vi "module information (FPGA interface).vi"(8 "error in":errorcluster, 10 "Module":u16, 11 "Refnum in":refnum<k20>) -> (0 "error out":errorcluster, 2 "Module Information":T1 {"product ID" format="%.0x"}, 3 "Refnum out":refnum<k20>)   [LabVIEW 2014, in "SMI.lvlib" / "C Series Module.lvclass"]
uses:
  C Series Module.lvclass
  Module/module information.ctl
  <vilib>/Utility/error.llb/Error Cluster From Error Code.vi
  <vilib>/rvi/errors/niLvFpgaAdjustHostInterfaceError.vi
  <vilib>/rvi/interface/nirviReadWriteControl/nirviReadWriteControl.xnode
  <vilib>/ErrorRing/Error Ring.xnode
  Module/Module.lvclass
  NiFpgaLv.dll
  <vilib>/rvi/interface/Simulation/niFpgaSimulationCallBeginRW.vi
  SMI.lvlib
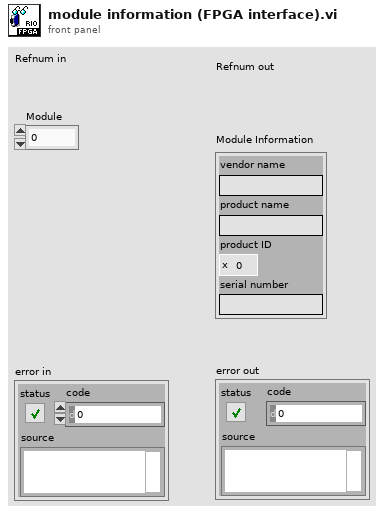
[diagram p1: front panel]
types:
  T1 = typedef "SMI.lvlib/Module.lvclass/module information.ctl" = cluster{"vendor name":string, "product name":string, "product ID":u16, "serial number":string}
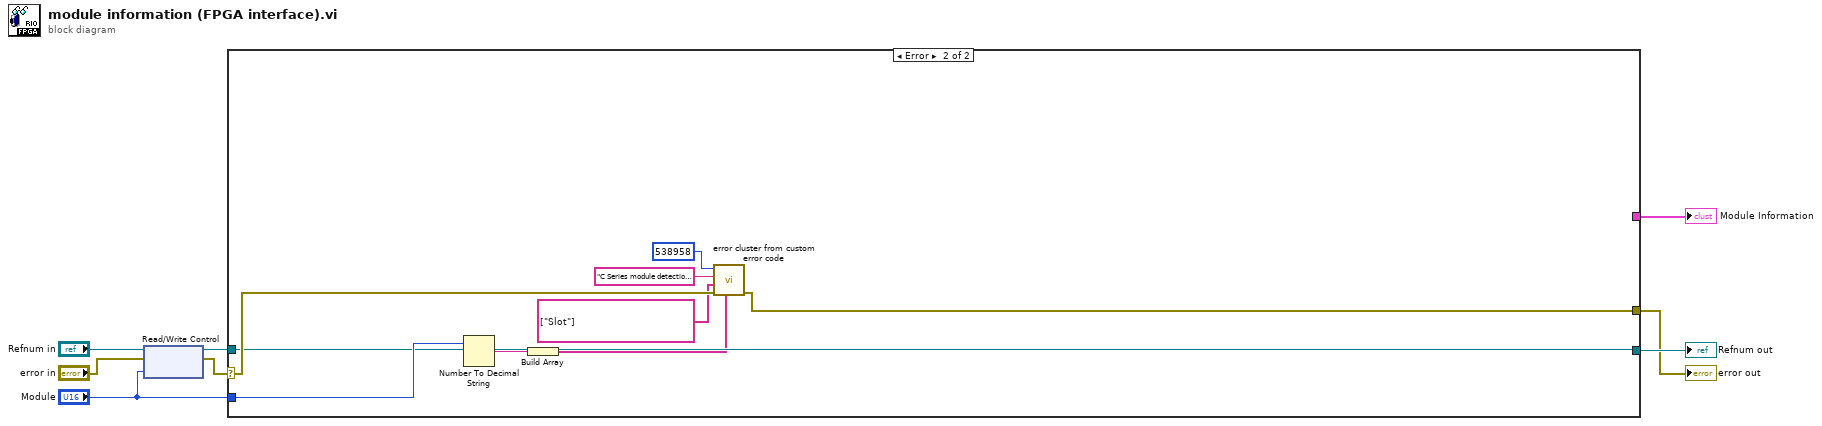
[diagram p0: block diagram]
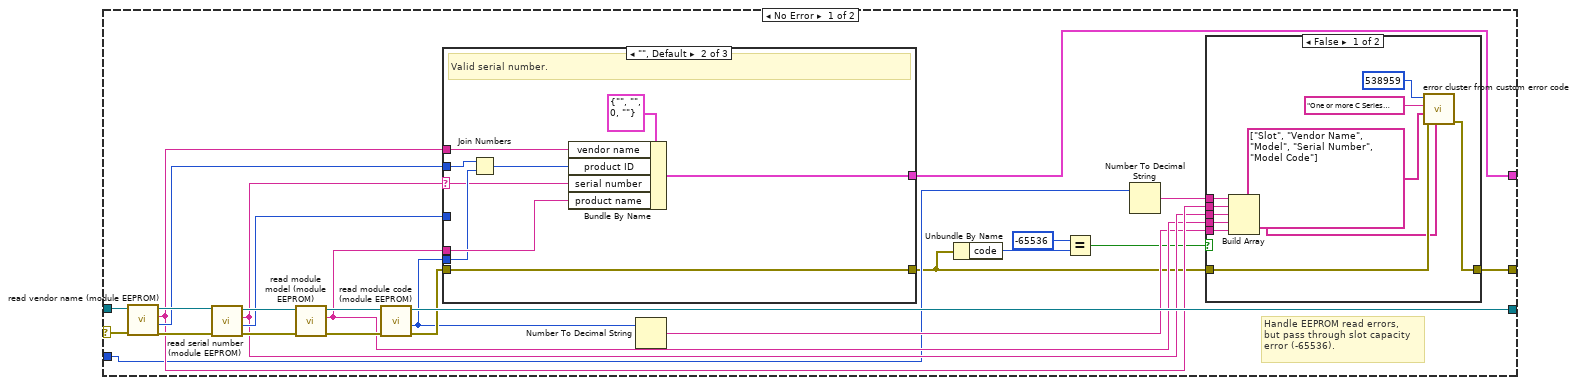
[diagram p2: hidden frame]
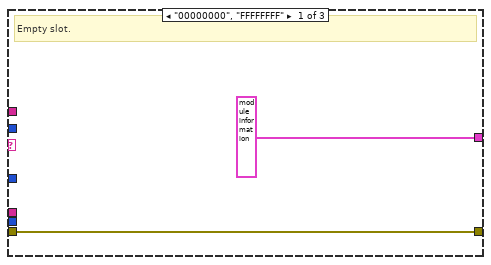
[diagram p4: hidden frame]
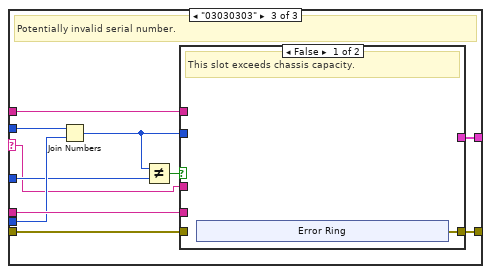
[diagram p5: hidden frame]
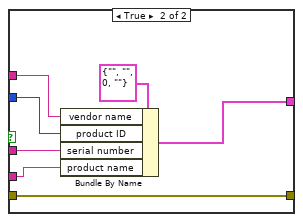
[diagram p6: hidden frame]
diagram:
  n1 = xnode "Read/Write Control"("FPGA VI Reference In"="Refnum in", "error in"="error in", "Module"="Module") -> ("FPGA VI Reference Out"=w8:refnum<k20>, "error out"=w2:errorcluster)
  n2 = case shown="Error" w2 {
    selector: w2 -> [w22 w88]
    tunnel: w8 -> [w29 w85]
    tunnel: [w26 w85] -> w5
    tunnel: [w20 w86] -> w4
    tunnel: [w21 _] -> w3
    tunnel: "Module" -> [w13 w87]
    frame No Error {
      # "Handle EEPROM read errors,\nbut pass through slot capacity\nerror (-65536)."
      n3 = call "read vendor name (module EEPROM).vi"("error in"=w22, "Refnum in"=w29) -> ("error out"=w30:errorcluster, "Vendor ID"=w25:u16, "Vendor Name"=w19:string, "Refnum out"=w31:refnum<k20>)  [unwired: 6 in]
      n4 = call "read serial number (module EEPROM).vi"("error in"=w30, "Refnum in"=w31) -> ("error out"=w33:errorcluster, "Serial Number"=w24:u32, "Serial Number String"=w18:string, "Refnum out"=w32:refnum<k20>)  [unwired: 6 in]
      n5 = call "read module model (module EEPROM).vi"("error in"=w33, "Refnum in"=w32) -> ("error out"=w28:errorcluster, "Module Model"=w17:string, "Refnum out"=w27:refnum<k20>)  [unwired: 7 in]
      n6 = call "read module code (module EEPROM).vi"("error in"=w28, "Refnum in"=w27) -> ("error out"=w23:errorcluster, "Module ID"=w16:u16, "Refnum out"=w26:refnum<k20>)  [unwired: 6 in, 1 out]
      n7 = case shown="\"\", Default" w18 {
        selector: w18 -> [_ w48 w58]
        tunnel: w19 -> [_ w56 w67]
        tunnel: w17 -> [_ w55 w66]
        tunnel: [T1 {"vendor name"="Not Present", "product name"="N/A", "product ID"=0, "serial number"="N/A"} ("cRIO Module Information") w54 w57] -> w21
        tunnel: w16 -> [_ w53 w65]
        tunnel: w25 -> [_ w52 w64]
        tunnel: w24 -> [_ _ w59]
        tunnel: w23 -> [w47 w49 w62]
        tunnel: [w47 w49 w61] -> w9
        frame "00000000", "FFFFFFFF" {
          # "Empty slot."
        }
        frame "", Default {
          # "Valid serial number."
          n8 = Join Numbers(hi=w52, lo=w53) -> ((hi.lo)=w50:u32)
          n9 = Bundle By Name(cluster=T1 {"vendor name"="", "product name"="", "product ID"=0, "serial number"=""} ("Module Information"), "vendor name"=w56, "product ID"=w50, "serial number"=w48, "product name"=w55) -> (w54:T1)
        }
        frame "03030303" {
          # "Potentially invalid serial number."
          n10 = Join Numbers(hi=w64, lo=w65) -> ((hi.lo)=w60:u32)
          n11 = Not Equal?(x=w60, y=w59) -> (x != y?=w63:bool)
          n12 = case shown="False" w63 {
            tunnel: w67 -> [_ w79]
            tunnel: w66 -> [_ w78]
            tunnel: [_ w77] -> w57
            tunnel: w58 -> [_ w76]
            tunnel: w60 -> [_ w74]
            tunnel: w62 -> [_ w73]
            tunnel: [w68 w73] -> w61
            frame False {
              # "This slot exceeds chassis capacity."
              n13 = xnode "Error Ring"() -> ("error out"=w68:errorcluster)
            }
            frame True {
              n14 = Bundle By Name(cluster=T1 {"vendor name"="", "product name"="", "product ID"=0, "serial number"=""} ("Module Information"), "vendor name"=w79, "product ID"=w74, "serial number"=w76, "product name"=w78) -> (w77:T1)
            }
          }
        }
      }
      n15 = Number To Decimal String(number=w16) -> (decimal integer string=w15:string)  [unwired: 1 in]
      n16 = Unbundle By Name(w9) -> ("code"=w12:i32)
      n17 = Equal?(x=-65536, y=w12) -> (x = y?=w10:bool)
      n18 = Number To Decimal String(number=w13) -> (decimal integer string=w14:string)  [unwired: 1 in]
      n19 = case shown="False" w10 {
        tunnel: [w44 w45] -> w20
        tunnel: w19 -> [w43 _]
        tunnel: w18 -> [w42 _]
        tunnel: w17 -> [w41 _]
        tunnel: w15 -> [w40 _]
        tunnel: w14 -> [w39 _]
        tunnel: w9 -> [w38 w45]
        frame False {
          n20 = Build Array(w39, w43, w42, w41, w40) -> (w35:string[])
          n21 = call "error cluster from custom error code.vi"("string values"=w35, "error in"=w38, "keys"=string[] ["Slot", "Vendor Name", "Model", "Serial Number", "Model Code"], "error message"="One or more C Series module properties could not be read from the EEPROM for the module in the chassis slot.", "custom error code (0)"=538959 ("error code (0)")) -> ("error out"=w44:errorcluster)  [unwired: 6 in]
        }
        frame True {
        }
      }
    }
    frame Error {
      n22 = Number To Decimal String(number=w87) -> (decimal integer string=w80:string)  [unwired: 1 in]
      n23 = Build Array(w80) -> (w82:string[])
      n24 = call "error cluster from custom error code.vi"("string values"=w82, "error in"=w88, "keys"=string[] ["Slot"], "error message"="C Series module detection failed for the chassis slot.", "custom error code (0)"=538958 ("error code (0)")) -> ("error out"=w86:errorcluster)  [unwired: 6 in]
    }
  }
  "Refnum out" <- w5
  "error out" <- w4
  "Module Information" <- w3
